vi "CANsub_Echo_C.vi"() -> ()   [LabVIEW 2021]
doc: "S5 echo (C client, direct wrapper calls): opens CH2 (C2, C4, C6, C2 after_ws), reads with TCP Read ? W13 C_Decode_RT, answers pings (C_Send_Pong), echoes harness test frames and reports their TX acks by UDP (Echo_Handle_Frames). Stop, peer close or an error ends the loop; C7 closes the channel. Reference for the API version."
uses:
  CANsub_C.lvlib
  common/CANsub_Common.lvlib
  common/Typedefs/REST_Phase.ctl
  Echo_Context.ctl
  Echo_Time_Store.ctl
  Echo_Counters.ctl
  common/Typedefs/CANsub_connection.ctl
  common/Typedefs/CANsub_Bit_Rates.ctl
  Echo_Config.ctl
panel:
  out "error out":errorcluster
  out "closed by device":bool
  out "nodelay":i32
  out "counters":T1
  in  "stop":bool
  in  "echo config":T2={"echo offset"=-256, "base id"=256, "report port"=5302} {"base id" format="%.0x"}
  in  "bit rates":T3={"nominal bit rate"=500000, "nominal sample point"=80.0, "data bit rate"=2000000, "data sample point"=80.0}
  in  "connection":T4={"host"="192.168.0.49", "channel"=2, "cert path"=path "/home/lvuser/cansub_root_cert.crt"}
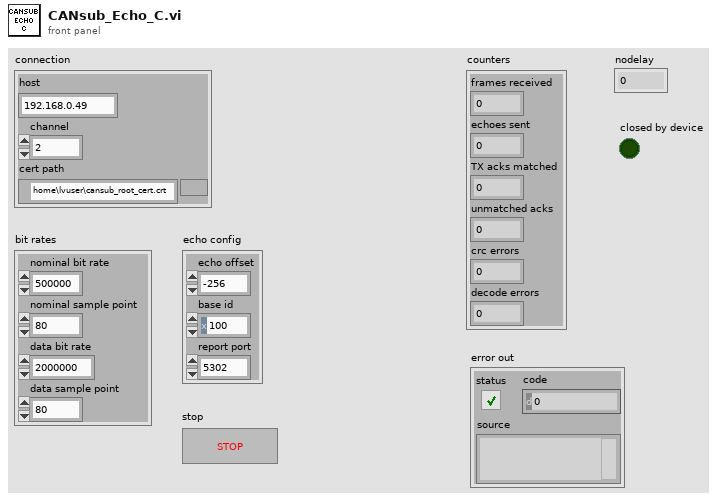
[diagram p1: front panel]
types:
  T1 = typedef "Echo_Counters.ctl" = cluster{"frames received":u32, "echoes sent":u32, "TX acks matched":u32, "unmatched acks":u32, "crc errors":u32, "decode errors":i32}
  T2 = typedef "Echo_Config.ctl" = cluster{"echo offset":i32, "base id":u32, "report port":u16}
  T3 = typedef "CANsub_Common.lvlib/CANsub_Bit_Rates.ctl" = cluster{"nominal bit rate":u32, "nominal sample point":dbl, "data bit rate":u32, "data sample point":dbl}
  T4 = typedef "CANsub_Common.lvlib/CANsub_connection.ctl" = cluster{"host":string, "channel":u8, "cert path":path}
  T5 = typedef "Echo_Time_Store.ctl" = cluster{"t_rx2_dev":dbl[], "t_rx2_lv":dbl[], "t_echo_send_lv":dbl[]}
  T6 = typedef "Echo_Context.ctl" = cluster{"TLS connection":refnum<k5>, "udp":refnum<k16>, "lv addr":u32, "report port":u16, "test lo":u32, "test hi":u32, "ack lo":u32, "ack hi":u32, "echo offset":i32}
  T7 = typedef "CANsub_Common.lvlib/REST_Phase.ctl" = enum16{"before_ws", "after_ws"}
  T8 = typedef "CANsub_Common.lvlib/Bit_Timing.ctl" = cluster{"brp":u16, "seg1":u16, "seg2":u16, "sjw":u16, "data brp":u16, "data seg1":u16, "data seg2":u16, "data sjw":u16}
  T9 = typedef "CANsub_C.lvlib/C_RX_Buffers.ctl" = cluster{"t_dev":dbl[], "ws":u8[], "id":u32[], "flags":u16[], "hdlc":u8[], "dlc":u8[], "data len":u8[], "data":u8[], "ping":u8[]}
  T10 = enum16{"Standard", "Buffered", "CRLF", "Immediate"}
  T11 = typedef "CANsub_C.lvlib/C_Decode_Result.ctl" = cluster{"n frames":i32, "peer close":bool, "ping len":i32, "crc errors":u32, "decode errors":i32}
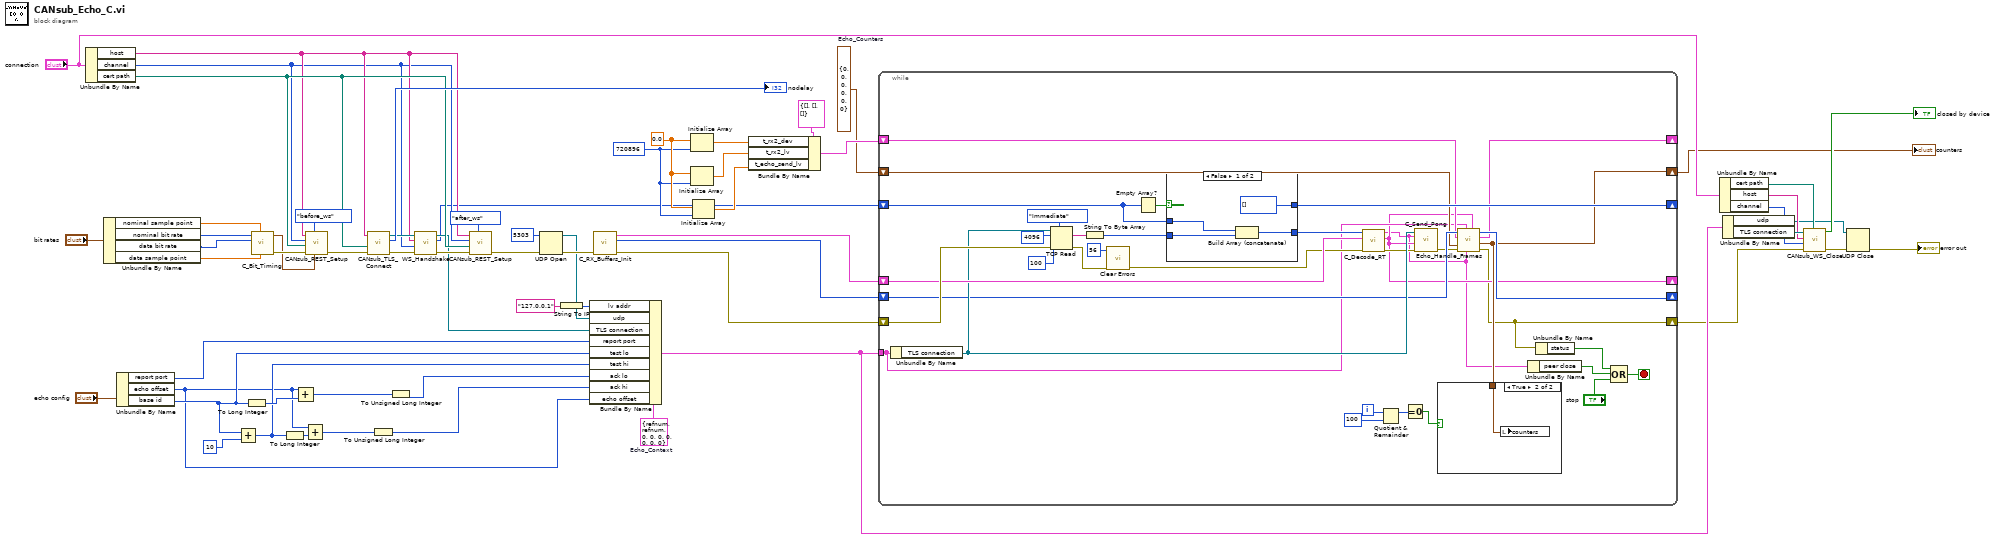
[diagram p0: block diagram]
diagram:
  w13 = T1 {"frames received"=0, "echoes sent"=0, "TX acks matched"=0, "unmatched acks"=0, "crc errors"=0, "decode errors"=0}  # Echo_Counters
  w23 = 720896 ("dimension size")
  w24 = 0.0
  w34 = T6 {"TLS connection"=refnum, "udp"=refnum, "lv addr"=0, "report port"=0, "test lo"=0, "test hi"=0, "ack lo"=0, "ack hi"=0, "echo offset"=0}  # Echo_Context
  n1 = Unbundle By Name("connection") -> ("host"=w41:string, "channel"=w40:u8, "cert path"=w44:path)
  n2 = Unbundle By Name("bit rates") -> ("nominal sample point"=w51:dbl, "nominal bit rate"=w50:u32, "data bit rate"=w49:u32, "data sample point"=w48:dbl)
  n3 = Unbundle By Name("echo config") -> ("report port"=w30:u16, "echo offset"=w25:i32, "base id"=w27:u32)
  n4 = Add(x=w27, y=u32 10) -> (x+y=w26:u32)
  n5 = To Long Integer(number=w27) -> (32bit integer=w38:i32)
  n6 = call "C_Bit_Timing.vi"("data sample point"=w48, "nominal sample point"=w51, "data bit rate"=w49, "nominal bit rate"=w50) -> ("error out"=w57:errorcluster, "Bit_Timing"=w47:T8)  [unwired: 4 in, 2 out]
  n7 = To Long Integer(number=w26) -> (32bit integer=w37:i32)
  n8 = Add(x=w25, y=w38) -> (x+y=w36:i32)
  n9 = Add(x=w25, y=w37) -> (x+y=w35:i32)
  n10 = call "CANsub_REST_Setup.vi"("bit timing"=w47, "phase"=REST_Phase."before_ws", "error in (no error)"=w57, "cert path"=w44, "channel"=w40, "host"=w41) -> ("error out"=w56:errorcluster)  [unwired: 4 in, 1 out]
  n11 = call "CANsub_TLS_Connect.vi"("error in (no error)"=w56, "cert path"=w44, "host"=w41) -> ("error out"=w55:errorcluster, "nodelay"=→"nodelay":i32, "TLS connection"=w45:refnum<k5>)  [unwired: 6 in]
  n12 = To Unsigned Long Integer(number=w35) -> (unsigned 32bit integer=w28:u32)
  n13 = To Unsigned Long Integer(number=w36) -> (unsigned 32bit integer=w29:u32)
  n14 = call "WS_Handshake.vi"("error in (no error)"=w55, "channel"=w40, "host"=w41, "TLS connection"=w45) -> ("error out"=w54:errorcluster, "leftover"=w15:u8[], "TLS connection out"=w33:refnum<k5>)  [unwired: 4 in, 1 out]
  n15 = call "CANsub_REST_Setup.vi"("phase"=REST_Phase."after_ws", "error in (no error)"=w54, "cert path"=w44, "channel"=w40, "host"=w41) -> ("error out"=w42:errorcluster)  [unwired: 5 in, 1 out]
  n16 = UDP Open(8:w42, 11:u16 5303 ("port")) -> (port=w32:refnum<k16>, 0:w52:errorcluster)  [unwired: 3 in, 1 out]
  n17 = String To IP(1:"127.0.0.1" ("name")) -> (0:w31:u32)
  n18 = Bundle By Name(cluster=w34, "lv addr"=w31, "udp"=w32, "TLS connection"=w33, "report port"=w30, "test lo"=w27, "test hi"=w26, "ack lo"=w29, "ack hi"=w28, "echo offset"=w25) -> (w11:T6)
  n19 = call "C_RX_Buffers_Init.vi"("error in (no error)"=w52) -> ("error out"=w18:errorcluster, "tx"=w16:u8[], "buffers"=w17:T9)  [unwired: 7 in, 1 out]
  n20 = Initialize Array(w24, w23) -> (w21:dbl[])
  n21 = Initialize Array(w24, w23) -> (w20:dbl[])
  n22 = Initialize Array(w24, w23) -> (w19:dbl[])
  n23 = Bundle By Name(cluster=T5 {"t_rx2_dev"=[], "t_rx2_lv"=[], "t_echo_send_lv"=[]} ("Echo_Time_Store"), "t_rx2_dev"=w21, "t_rx2_lv"=w20, "t_echo_send_lv"=w19) -> (w14:T5)
  n24 = while {
    shift-right: [w74] -> _
    shift-left: w14 -> [w78]
    shift-right: [w69] -> w1
    shift-left: w13 -> [w77]
    shift-right: [w87] -> _
    shift-left: w15 -> [w86]
    shift-right: [w66] -> _
    shift-left: w17 -> [w84]
    shift-right: [w75] -> _
    shift-left: w16 -> [w80]
    shift-right: [w64] -> w5
    shift-left: w18 -> [w93]
    tunnel: w11 -> [w76]
    i -> [w73]
    stop <- w68 stop-if-true
    n25 = Unbundle By Name(w76) -> ("TLS connection"=w82:refnum<k5>)
    n26 = TCP Read(connection ID=w82, bytes to read=4096, error in (no error)=w93, 7:T10."Immediate" ("mode (standard)"), 9:100 ("timeout ms (25000)")) -> (data out=w90:string, error out=w91:errorcluster)  [unwired: 1 out]
    n27 = String To Byte Array(string=w90) -> (unsigned byte array=w88:u8[])
    n28 = call <vilib>:"Clear Errors.vi"("error in (no error)"=w91, "specific error code to clear (0: all)"=56) -> ("error out"=w83:errorcluster)  [unwired: 4 in, 1 out]
    n29 = Empty Array?(array=w86) -> (empty?=w89:bool)
    n30 = case shown="False" w89 {
      tunnel: w88 -> [w101 w102]
      tunnel: [u8[] [] ("leftover") w103] -> w87
      tunnel: w86 -> [w100 w103]
      tunnel: [w99 w102] -> w85
      frame False {
        n31 = Build Array (concatenate)(w100, w101) -> (w99:u8[])
      }
      frame True {
      }
    }
    n32 = call "C_Decode_RT.vi"("error in (no error)"=w83, "buffers in"=w84, "bytes in"=w85) -> ("error out"=w81:errorcluster, "buffers out"=w66:T9, "result"=w65:T11)  [unwired: 6 in]
    n33 = Quotient & Remainder(x=w73, y=100) -> (x-y*floor(x/y)=w71:i32)  [unwired: 1 out]
    n34 = Equal To 0?(x=w71) -> (x = 0?=w70:bool)
    n35 = call "C_Send_Pong.vi"("error in (no error)"=w81, "buffers"=w66, "result"=w65, "TLS connection"=w82) -> ("error out"=w79:errorcluster)  [unwired: 7 in]
    n36 = call "Echo_Handle_Frames.vi"("buffers"=w66, "result"=w65, "context"=w76, "error in (no error)"=w79, "counters in"=w77, "time store in"=w78, "tx in"=w80) -> ("error out"=w64:errorcluster, "counters out"=w69:T1, "time store out"=w74:T5, "tx out"=w75:u8[])  [unwired: 1 in]
    n37 = case shown="True" w70 {
      tunnel: w69 -> [_ w97]
      frame False {
      }
      frame True {
        n38 = local write "counters"(w97) -> ()
      }
    }
    n39 = Unbundle By Name(w65) -> ("peer close"=w63:bool)
    n40 = Unbundle By Name(w64) -> ("status"=w62:bool)
    n41 = Compound Arithmetic op=OR(w62, w63, "stop") -> (w68:bool)
  }
  "counters" <- w1
  n42 = Unbundle By Name("connection") -> ("cert path"=w8:path, "host"=w7:string, "channel"=w6:u8)
  n43 = Unbundle By Name(w11) -> ("udp"=w3:refnum<k16>, "TLS connection"=w10:refnum<k5>)
  n44 = call "CANsub_WS_Close.vi"("cert path"=w8, "error in (no error)"=w5, "channel"=w6, "host"=w7, "TLS Connection"=w10) -> ("error out"=w12:errorcluster, "closed by device"=→"closed by device":bool)  [unwired: 5 in]
  n45 = UDP Close(connection ID=w3, 8:w12) -> (error out=→"error out":errorcluster)  [unwired: 1 out]
